vi "optical_grab2.vi"() -> ()   [LabVIEW 2025]
uses:
  <vilib>/vision/driver/NI_Vision_Acquisition_Software.lvlib
  <resource>/objmgr/imaqdx.rc
panel:
  out "Time bw Frames":u32
  out "max value":u16
  out "Image Pixels (U16)":u16[][](array[numeric])
  out "Image Preview":T1(plugin-control)
  out "error out":errorcluster
  out "FPS":u32
  in  "Output Folder":path=path "../data/raw/test_6"
  in  "Stop":bool
  in  "Camera Name":refnum<k21> caption="IMAQdx Session"
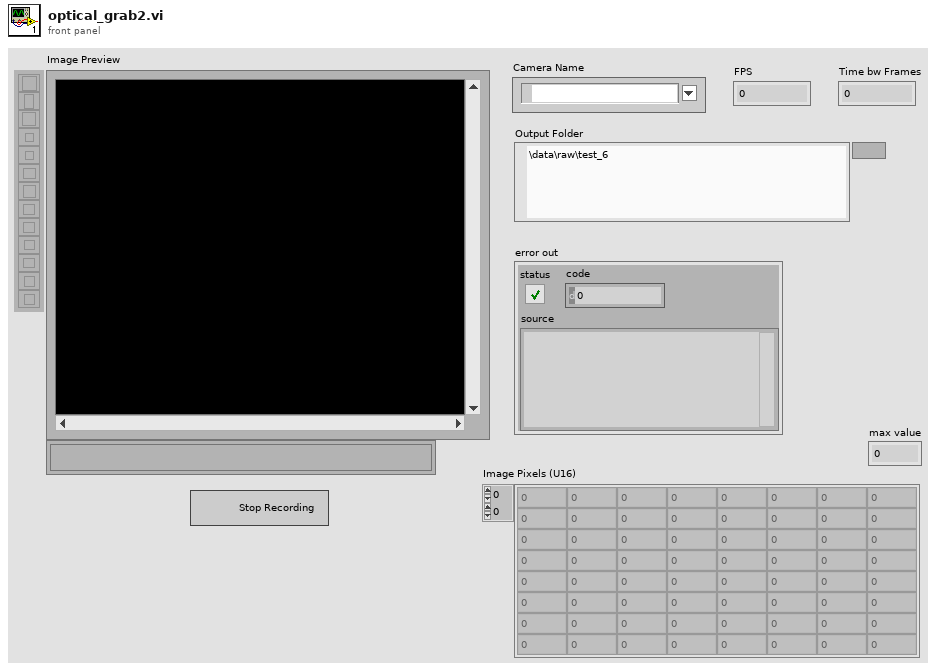
[diagram p1: front panel]
types:
  T1 = typedef "IMAQ Image.ctl" = refnum<image>
  T2 = typedef "Image Type" = u32
  T3 = typedef "IMAQdx.ctl" = refnum<k21>
  T4 = enum16{"big-endian, network order", "native, host order", "little-endian"}
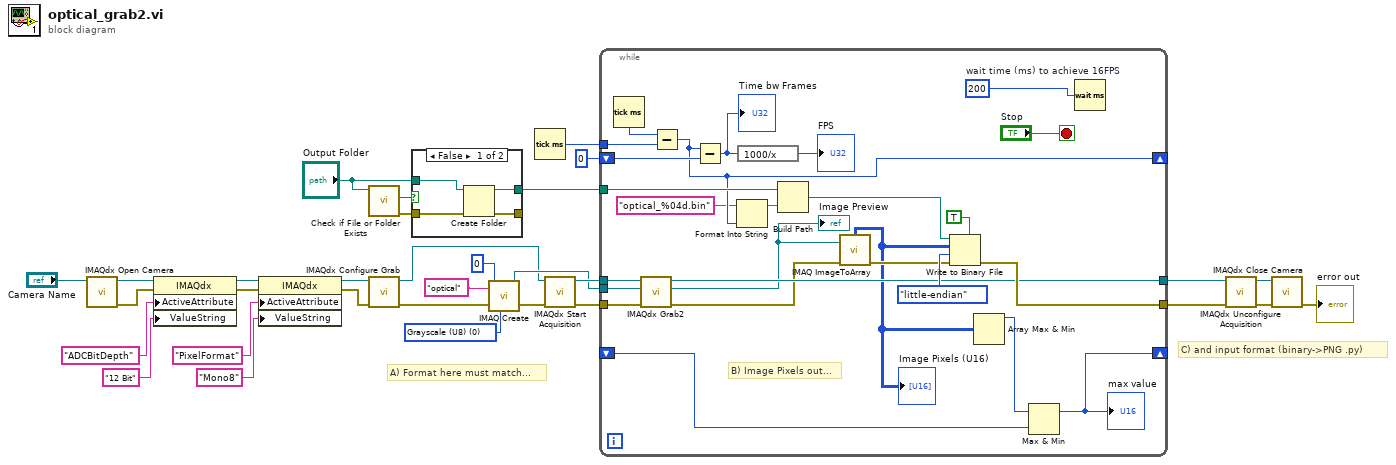
[diagram p0: block diagram]
diagram:
  w23 = T2 0 items=["Grayscale (U8)", "Grayscale (I16)", "Grayscale (SGL)", "Complex (CSG)", "RGB (U32)", "HSL (U32)", "RGB (U64)", "Grayscale (U16)"] ("Image Type")
  # "C) and input format (binary->PNG .py)"
  # "A) Format here must match..."
  n1 = call <vilib>:"IMAQdx Open Camera.vi"("Session In"="Camera Name") -> ("error out"=w19:errorcluster, "Session Out"=w20:T3)  [unwired: 9 in]
  n2 = property class="IMAQdx"(reference=w20, error in=w19, "ActiveAttribute"="ADCBitDepth", "ValueString"="12 Bit") -> (reference out=w6:T3, error out=w4:errorcluster)
  n3 = property class="IMAQdx"(reference=w6, error in=w4, "ActiveAttribute"="PixelFormat", "ValueString"="Mono8" ("ActiveAttribute")) -> (reference out=w5:T3, error out=w3:errorcluster)
  n4 = call <vilib>:"Check if File or Folder Exists.vi"("path"="Output Folder") -> ("error out"=w29:errorcluster, "file or folder exists?"=w31:bool)  [unwired: 8 in, 1 out]
  n5 = call <vilib>:"IMAQdx Configure Grab.vi"("error in"=w3, "Session In"=w5) -> ("error out"=w10:errorcluster, "Session Out"=w9:T3)  [unwired: 8 in]
  n6 = case shown="False" w31 {
    tunnel: "Output Folder" -> [w35 w37]
    tunnel: [w34 w37] -> w28
    tunnel: w29 -> [w33 w36]
    tunnel: [w32 w36] -> _
    frame False {
      n7 = Create Folder(path (use dialog)=w35, error in=w33) -> (created path=w34:path, error out=w32:errorcluster)  [unwired: 1 in, 1 out]
    }
    frame True {
    }
  }
  n8 = call "IMAQ Create"("Border Size"=0, "Image Name"="optical", "Image Type"=w23, "error in (no error)"=w10) -> ("New Image"=w13:T1, "error out"=w12:errorcluster)  [unwired: 1 in]
  n9 = Tick Count (ms)() -> (millisecond timer value=w27:u32)
  n10 = call <vilib>:"IMAQdx Start Acquisition.vi"("error in"=w12, "Session In"=w9) -> ("error out"=w11:errorcluster, "Session Out"=w21:T3)  [unwired: 8 in]
  n11 = while {
    tunnel: w28 -> [w63]
    tunnel: w27 -> [w61]
    shift-right: [w59] -> _
    shift-left: u32 0 -> [w60]
    tunnel: w21 -> [w55]
    tunnel: w13 -> [w54]
    tunnel: w11 -> [w53]
    tunnel: [w47] -> w18
    tunnel: [w51] -> w15
    shift-right: [w41] -> _
    shift-left: _ -> [w42]
    stop <- "Stop" stop-if-true
    w40 = u32 200  # wait time (ms) to achieve 16FPS
    # "B) Image Pixels out..."
    n12 = Tick Count (ms)() -> (millisecond timer value=w62:u32)
    n13 = call <vilib>:"IMAQdx Grab2.vi"("error in"=w53, "Image In"=w54, "Session In"=w55) -> ("error out"=w45:errorcluster, "Image Out"=w46:T1, "Session Out"=w47:T3)  [unwired: 5 in, 1 out]
    "Image Preview" <- w46
    n14 = Subtract(x=w62, y=w61) -> (x-y=w59:u32)
    n15 = Subtract(x=w59, y=w60) -> (x-y=w39:u32)
    "Time bw Frames" <- w39
    n16 = Format Into String(format string="optical_%04d.bin", w59) -> (resulting string=w58:string)  [unwired: 2 in, 1 out]
    n17 = expression code="1000/x"(w39) -> (→"FPS":u32)
    n18 = Build Path(base path=w63, name or relative path=w58) -> (appended path=w52:path)
    n19 = call "IMAQ ImageToArray"("error in (no error)"=w45, "Image"=w46) -> ("error out"=w44:errorcluster, "Image Pixels (U8)"=w38:u8[][])  [unwired: 2 in, 3 out]
    "Image Pixels (U16)" <- w38
    n20 = Write to Binary File(file (use dialog)=w52, data=w38, error in=w44, 5:TRUE, 9:T4."little-endian" ("byte order (0:big-endian, network order)")) -> (error out=w51:errorcluster)  [unwired: 1 in, 2 out]
    n21 = Array Max & Min(array=w38) -> (max value=w43:u8)  [unwired: 3 out]
    n22 = Max & Min(x=w43, y=w42) -> (max(x,y)=w41:u8)  [unwired: 1 out]
    "max value" <- w41
    n23 = Wait (ms)(milliseconds to wait=w40) -> ()  [unwired: 1 out]
  }
  n24 = call <vilib>:"IMAQdx Unconfigure Acquisition.vi"("error in"=w15, "Session In"=w18) -> ("error out"=w16:errorcluster, "Session Out"=w17:T3)  [unwired: 8 in]
  n25 = call <vilib>:"IMAQdx Close Camera.vi"("error in"=w16, "Session In"=w17) -> ("error out"=→"error out":errorcluster)  [unwired: 9 in]
